vi "Add Timing Section.vi"(8 "error in":errorcluster, 11 "custom device ref":T1 format="%.0x") -> (0 "error out":errorcluster, 2 "timing":T1 format="%.0x", 3 "custom device ref out":T1 format="%.0x")   [LabVIEW 2020, in "AIM ARINC 429 Scripting.lvlib"]
uses:
  AIM ARINC 429 Scripting.lvlib
  <vilib>/NI VeriStand/Custom Device API/Custom Device Item Ref.ctl
  <vilib>/NI VeriStand/Custom Device API/Custom Device Channel.ctl
  <vilib>/NI VeriStand/Custom Device API/Custom Device Channel Type.ctl
  Constants.vi
  <vilib>/NI VeriStand/Custom Device API/Custom Device API.lvlib
  <vilib>/NI VeriStand/Custom Device Offline API/Custom Device Offline API.lvlib
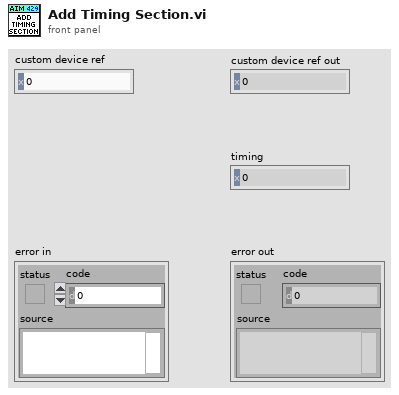
[diagram p1: front panel]
types:
  T1 = typedef "Custom Device API.lvlib/Custom Device Item Ref.ctl" = u64
  T2 = typedef "Custom Device API.lvlib/Custom Device Channel.ctl" = cluster{"Type":T3, "Units":string, "Default Value":dbl, "Faultable":bool, "Scalable":bool}
  T3 = typedef "Custom Device API.lvlib/Custom Device Channel Type.ctl" = enum16{"Input", "Output"}
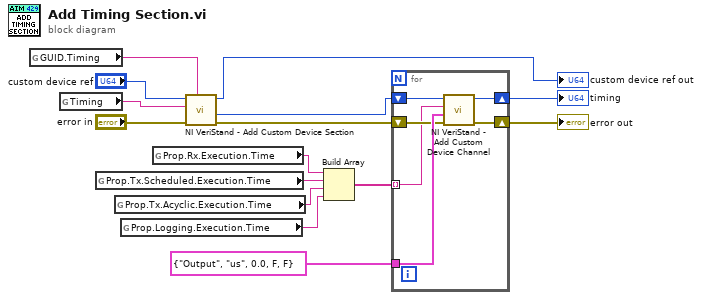
[diagram p0: block diagram]
diagram:
  n1 = global read "Constants.vi" "GUID.Timing"() -> (w13:string)
  n2 = global read "Constants.vi" "Timing"() -> (w12:string)
  n3 = global read "Constants.vi" "Prop.Tx.Scheduled.Execution.Time"() -> (w3:string)
  n4 = global read "Constants.vi" "Prop.Tx.Acyclic.Execution.Time"() -> (w2:string)
  n5 = global read "Constants.vi" "Prop.Logging.Execution.Time"() -> (w1:string)
  n6 = global read "Constants.vi" "Prop.Rx.Execution.Time"() -> (w4:string)
  n7 = call <vilib>:"NI VeriStand - Add Custom Device Section.vi"("GUID (Default Section)"=w13, "error in (no error)"="error in", "Section Name"=w12, "Parent Ref in"="custom device ref") -> ("error out"=w9:errorcluster, "Section Ptr"=w7:T1, "Parent Ref out"=→"custom device ref out":T1)  [unwired: 4 in, 1 out]
  n8 = Build Array(w4, w3, w2, w1) -> (w10:string[])
  n9 = for {
    tunnel: T2 {"Type"=enum."Output", "Units"="us", "Default Value"=0.0, "Faultable"=FALSE, "Scalable"=FALSE} ("Channel") -> [w20]
    shift-right: [w17] -> w5
    shift-left: w7 -> [w21]
    shift-right: [w18] -> w8
    shift-left: w9 -> [w19]
    tunnel: w10 -> [w16] mode=indexing
    n10 = call <vilib>:"NI VeriStand - Add Custom Device Channel.vi"("error in (no error)"=w19, "Channel"=w20, "Channel Name"=w16, "Parent Ref in"=w21) -> ("error out"=w18:errorcluster, "Parent Ref out"=w17:T1)  [unwired: 4 in, 2 out]
  }
  "error out" <- w8
  "timing" <- w5
